vi "VIH HelpGen - Replace ProductInfo Keywords in String.vi"(7 "Coded to HTML (F)":bool, 8 "Init (F)":bool, 10 "PINF Prefix":string, 11 "String in":string) -> (3 "String out":string)   [LabVIEW 2014]
doc: "::: VI Helpeks :::\nCopyright (c) 2000-2026 Konstantin Shifershteyn. All rights reserved."
panel:
  # "VI Helpeks\nCopyright (c) 2012-2026 Konstantin Shifershteyn"
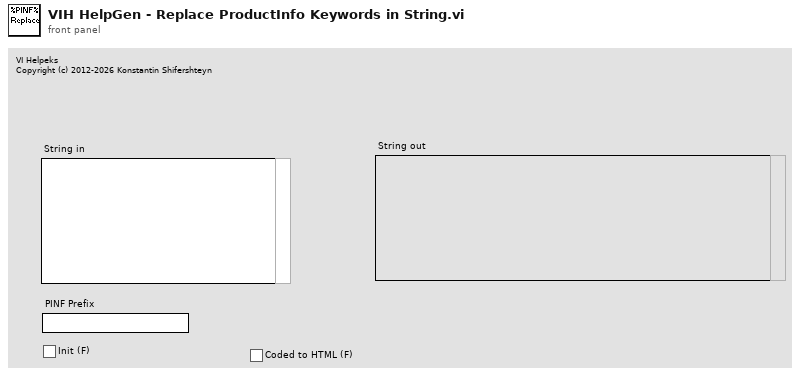
[diagram p1: front panel]
types:
  T1 = enum16{"none", "LV description", "VH minimum", "VH extended"}
  T2 = typedef "VIH HelpGen Typedef - Product Info Cluster.ctl" = cluster{"ProductName":string, "Version":string, "Author":string, "Company":string, "Copyright":string, "Website":string, "Email":string, "AddInfo":string}
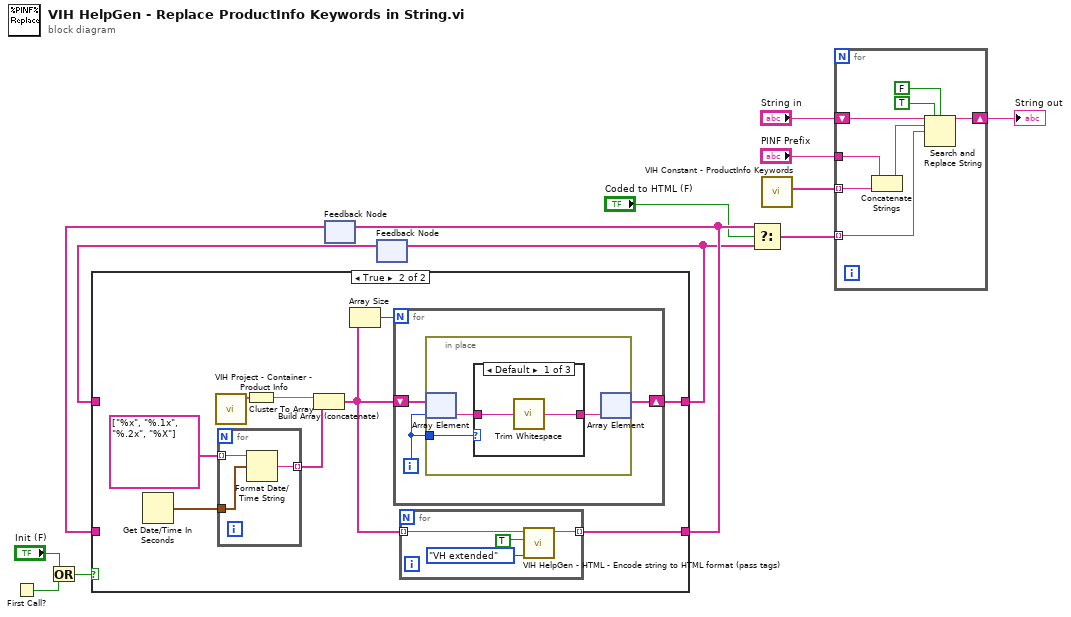
[diagram p0: block diagram]
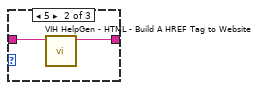
[diagram p3: hidden frame]
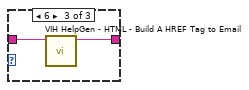
[diagram p4: hidden frame]
diagram:
  n1 = First Call?() -> (First Call?: T/F=w9:bool)
  n2 = Or(x="Init (F)", y=w9) -> (x .or. y?=w8:bool)
  n3 = feedback #1() -> (w5:string[])  [unwired: 1 in]
  n4 = feedback #2() -> (w7:string[])  [unwired: 1 in]
  n5 = case shown="True" w8 {
    tunnel: [w15 w22] -> w3
    tunnel: w7 -> [w15 _]
    tunnel: [w14 w16] -> w4
    tunnel: w5 -> [w14 _]
    frame False {
    }
    frame True {
      n6 = Get Date/Time In Seconds() -> (seconds since 1Jan1904=w18:timestamp)
      n7 = call "VIH Project - Container - Product Info.vi"() -> ("Product Info out"=w24:T2)  [unwired: 11 in]
      n8 = for {
        tunnel: string[] ["%x", "%.1x", "%.2x", "%X"] -> [w31] mode=indexing
        tunnel: [w30] -> w19 mode=indexing
        tunnel: w18 -> [w29]
        n9 = Format Date/Time String(time format string (%c)=w31, seconds (now)=w29) -> (date/time string=w30:string)  [unwired: 1 in]
      }
      n10 = Cluster To Array(cluster=w24) -> (array=w20:string[])
      n11 = Build Array (concatenate)(w20, w19) -> (w17:string[])
      n12 = Array Size(array=w17) -> (size(s)=w23:i32)
      n13 = for {
        N: w23 -> [_]
        shift-right: [w32] -> w22
        shift-left: w17 -> [w34]
        i -> [w33]
        n14 = in-place {
          in-place-border: w33 -> [w37]
          n15 = in-place-array #3(w34, w33) -> (w35:string)
          n16 = case shown="Default" w37 {
            tunnel: [w38 w41 w42] -> w36
            tunnel: w35 -> [w39 w40 w43]
            frame Default {
              n17 = call <vilib>:"Trim Whitespace.vi"("string"=w39) -> ("trimmed string"=w38:string)  [unwired: 1 in]
            }
            frame 5 {
              n18 = call "VIH HelpGen - HTML - Build A HREF Tag to Website.vi"("URL"=w40) -> ("HTML tag"=w41:string)  [unwired: 10 in]
            }
            frame 6 {
              n19 = call "VIH HelpGen - HTML - Build A HREF Tag to Email.vi"("Email address"=w43) -> ("HTML tag"=w42:string)  [unwired: 10 in]
            }
          }
          n20 = in-place-array #3(w36) -> (w32:string[])  [unwired: 1 out]
        }
      }
      n21 = for {
        tunnel: w17 -> [w26] mode=indexing
        tunnel: [w25] -> w16 mode=indexing
        n22 = call "VIH HelpGen - HTML - Encode string to HTML format (pass tags).vi"("HTML Tagset allowed"=T1."VH extended", "Reject CR (F)"=TRUE, "string"=w26) -> ("HTML string"=w25:string)  [unwired: 8 in]
      }
    }
  }
  n23 = feedback-in #1(w4) -> ()
  n24 = feedback-in #2(w3) -> ()
  n25 = Select(t=w4, s="Coded to HTML (F)", f=w3) -> (s? t:f=w1:string[])
  n26 = call "VIH Constant - ProductInfo Keywords.vi"() -> ("ProductInfo keywords"=w11:string[])  [unwired: 10 in, 1 out]
  n27 = for {
    shift-right: [w48] -> w12
    shift-left: "String in" -> [w51]
    tunnel: w11 -> [w46] mode=indexing
    tunnel: w1 -> [w47] mode=indexing
    tunnel: "PINF Prefix" -> [w45]
    n28 = Concatenate Strings(w45, w46) -> (w44:string)
    n29 = Search and Replace String(replace all?=TRUE, case sensitive?=FALSE ("ignore case? (F)"), input string=w51, search string=w44, replace string=w47) -> (result string=w48:string)  [unwired: 3 in, 3 out]
  }
  "String out" <- w12
